vi "01a-add_two_numbers.vi"() -> ()   [LabVIEW 2018, in "LV2Julia_examples.lvlib"]
uses:
  LV2Julia_examples.lvlib
  LV2Julia_core/VIs/Server or client state.ctl
  LV2Julia_core/VIs/detailed error info.ctl
  LV2Julia_core/VIs/StackFrame.ctl
  LV2Julia_core/VIs/Commands.ctl
  a521f879-d34e-4576-958d-ff4dfcea3e86.vi
  be4745b6-8471-45fc-b8a0-8968ce92ea4b.vi
  5a89c37d-8165-4bab-9232-2165bf484997.vi
  <vilib>/Utility/High Resolution Relative Seconds.vi
  be4745b6-8471-45fc-b8a0-8968ce92ea4b.vi/01ce1741-ea78-47f8-98ed-e79163fb1a9b.vi
  be4745b6-8471-45fc-b8a0-8968ce92ea4b.vi/01ce1741-ea78-47f8-98ed-e79163fb1a9b.vi/cc3cf2af-bc3b-4fb6-855b-7562c4d0bfeb.vi
  be4745b6-8471-45fc-b8a0-8968ce92ea4b.vi/01ce1741-ea78-47f8-98ed-e79163fb1a9b.vi/c77cecd8-10de-4d46-bc1c-57302a887fda.vi
  be4745b6-8471-45fc-b8a0-8968ce92ea4b.vi/01ce1741-ea78-47f8-98ed-e79163fb1a9b.vi/2cafb1dd-d397-4b79-911a-06d102936120.vi
  LV2Julia_core/VIs/jl-scripts path.vi
  LV2Julia_core/VIs/check ID validity.vi
  LV2Julia_core/VIs/bindata_descr to JSON.vi
  LV2Julia_core/VIs/check cluster field names.vi
  LV2Julia_core/VIs/concat JSON.vi
  LV2Julia_core/VIs/build request.vi
  LV2Julia_core/VIs/Parse server response.vi
  LV2Julia_core/VIs/log jl exceptions.vi
  LV2Julia_core/LV2Julia_core.lvlib
panel:
  out "call duration (ms)":dbl format="%#.2f"
  in  "summands":cluster{"x":dbl, "y":dbl}={"x"=2.0, "y"=2.0}
  in  "next":bool
  out "x+y":dbl=nan
  out "detailed error info":T1
  out "current error":errorcluster
  out "final error":errorcluster
  out "short err code":u8
  in  "stop":bool
  out "ZMQ timeout":bool
  out "Julia script file path":path
  out "temporary script path":path
  out "Jl Server state":T3
  # "After the Julia server started (Jl Server state changed to \"running\", also see the Windows command line window), click onto  Next to get the calculation result. Click onto stop to  stop this VI as well as the Julia server.\n\nNote that the first call of a Julia function may take a fraction of second due to JIT compilation"
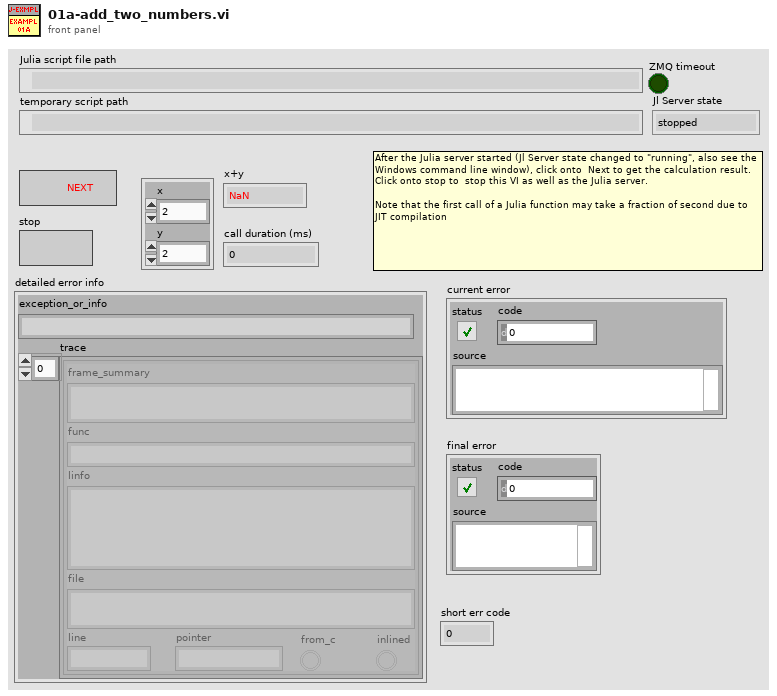
[diagram p1: front panel]
types:
  T1 = typedef "LV2Julia_core.lvlib/detailed error info.ctl" = cluster{"exception_or_info":string, "trace":T2[]}
  T2 = typedef "LV2Julia_core.lvlib/StackFrame.ctl" = cluster{"frame_summary":string, "func":string, "linfo":string, "file":string, "line":i32, "pointer":u64, "from_c":bool, "inlined":bool}
  T3 = typedef "LV2Julia_core.lvlib/Server or client state.ctl" = enum16{"stopped", "running", "unknown"}
  T4 = typedef "LV2Julia_core.lvlib/Commands.ctl" = enum16{"Start Jl-server & Init LV-client", "Send request & Get response ", "Stop Jl-server & Cleanup LV-client", "Cleanup LV-client", "Start Jl-server", "Stop Jl-server", "Init LV-Client", "Cleanup LV-Client", "(not allowed)", "Set LV Client state", "Set Jl Server state", "set ZMQ timeout", "read ZMQ timeout", "read-out state"}
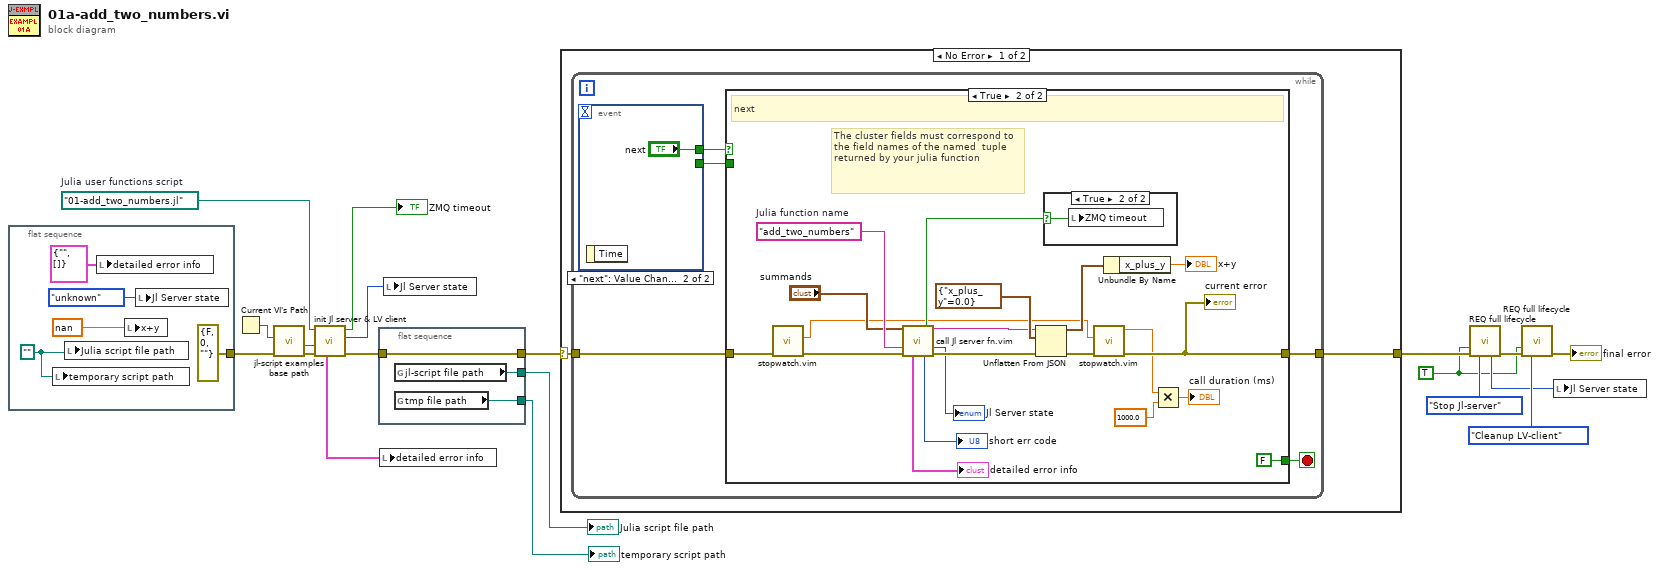
[diagram p0: block diagram]
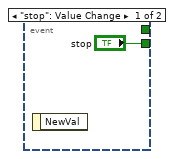
[diagram p2: hidden frame]
diagram:
  w10 = path "01-add_two_numbers.jl"  # Julia user functions script
  w9 = TRUE ("Force command")
  n1 = flat-sequence {
    tunnel: [errorcluster {"status"=FALSE, "code"=0, "source"=""} ("error in (no error)")] -> w5
    frame #0 {
      w20 = path ""
      n2 = local write "temporary script path"(w20) -> ()
      n3 = local write "Julia script file path"(w20) -> ()
      n4 = local write "detailed error info"(T1 {"exception_or_info"="", "trace"=[]} ("detailed error info")) -> ()
      n5 = local write "x+y"(nan ("Server response")) -> ()
      n6 = local write "Jl Server state"(Server_or_client_state."unknown" ("Jl Server state out")) -> ()
    }
  }
  n7 = Current VI's Path() -> (path=w2:path)
  n8 = call "jl-script examples base path.vi"("error in (no error)"=w5, "calling example VI path"=w2) -> ("error out"=w4:errorcluster, "jl-script-examples base path"=w3:path)  [unwired: 8 in]
  n9 = call "init Jl server & LV client.vi"("error in (no error)"=w4, "Base path (not a path)"=w3, "Julia user functions script"=w10) -> ("error out"=w7:errorcluster, "Jl Server state out"=w6:T3, "timeout?"=→"ZMQ timeout":bool, "detailed error info"=w1:T1)  [unwired: 3 in, 2 out]
  n10 = flat-sequence {
    tunnel: [w27] -> w14
    tunnel: w7 -> [w27]
    tunnel: [w26] -> w12
    tunnel: [w25] -> w13
    frame #0 {
      n11 = global read "jl-scripts path.vi" "jl-script file path"() -> (w26:path)
      n12 = global read "jl-scripts path.vi" "tmp file path"() -> (w25:path)
    }
  }
  n13 = local write "detailed error info"(w1) -> ()
  n14 = local write "Jl Server state"(w6) -> ()
  n15 = case shown="No Error" w14 {
    selector: w14 -> [w28 w60]
    tunnel: [w29 w60] -> w19
    frame No Error {
      n16 = while {
        tunnel: w28 -> [w33]
        tunnel: [w34] -> w29
        stop <- w31 stop-if-true
        n17 = event shown="[1] \"next\": Value Change" {
          selector: _ -> [_ _]
          dyn-events: _ -> [_ _]
          timeout: _ -> [_ _]
          tunnel: [_ "next"] -> w32
          tunnel: ["stop" _] -> w30
          event "stop": Value Change {
            n18 = event-data() -> ()  [unwired: 1 in, 1 out]
          }
          event "next": Value Change {
            n19 = event-data() -> ()  [unwired: 1 in, 1 out]
          }
        }
        n20 = case shown="True" w32 {
          tunnel: [w38 w41] -> w34
          tunnel: w33 -> [w38 w45]
          tunnel: [w37 FALSE ("stop this VI only")] -> w31
          tunnel: w30 -> [w37 _]
          frame False {
            # "stop"
          }
          frame True {
            w55 = "add_two_numbers"  # Julia function name
            # "The cluster fields must correspond to the field names of the named  tuple returned by your julia function"
            # "next"
            n21 = call "stopwatch.vim"("anything in"=w45) -> ("copy of anything out"=w44:errorcluster, "current timepoint"=w40:dbl)  [unwired: 8 in, 1 out]
            n22 = call "call Jl server fn.vim"("Arguments 1"="summands", "fun2call"=w55, "error in (no error)"=w44) -> ("timeout?"=w52:bool, "JSON received"=w49:string, "Jl Server state out"=→"Jl Server state":T3, "detailed error info"=→"detailed error info":T1, "return code"=→"short err code":u8, "error out"=w51:errorcluster)  [unwired: 6 in, 1 out]
            n23 = Unflatten From JSON(JSON string=w49, type and defaults=cluster{"x_plus_y":dbl} {"x_plus_y"=0.0} ("parsed response"), error in (no error)=w51) -> (value=w43:cluster{"x_plus_y":dbl}, error out=w42:errorcluster)  [unwired: 4 in]
            n24 = case shown="True" w52 {
              selector: w52 -> [_ w59]
              frame False {
              }
              frame True {
                n25 = local write "ZMQ timeout"(w59) -> ()
              }
            }
            n26 = call "stopwatch.vim"("anything in"=w42, "prev timepoint (0)"=w40) -> ("copy of anything out"=w41:errorcluster, "delta t (s)"=w39:dbl)  [unwired: 7 in, 1 out]
            "current error" <- w41
            n27 = Unbundle By Name(w43) -> ("x_plus_y"=→"x+y":dbl)
            n28 = Multiply(x=w39, y=1000.0) -> (x*y=→"call duration (ms)":dbl)
          }
        }
      }
    }
    frame Error {
    }
  }
  n29 = call "REQ full lifecycle.vi"("Force command"=w9, "error in"=w19, "command"=Commands."Stop Jl-server") -> ("Jl Server state out"=w11:T3, "error out"=w17:errorcluster)  [unwired: 6 in, 5 out]
  n30 = call "REQ full lifecycle.vi"("Force command"=w9, "error in"=w17, "command"=Commands."Cleanup LV-client") -> ("error out"=→"final error":errorcluster)  [unwired: 6 in, 6 out]
  n31 = local write "Jl Server state"(w11) -> ()
  "temporary script path" <- w13
  "Julia script file path" <- w12
